vi "fake tool unwired error.vi"(11 "json":string) -> (3 "count":i32)   [LabVIEW 2020, in "MCP Server tests.lvlib"]
doc: "Test fixture tool: counts the items of the JSON object json. The parse error of a json that is not an object appears on an unwired error output, and the VI has automatic error handling enabled, so that a server which runs it without switching that off opens LabVIEW's modal error dialog."
uses:
  MCP Server tests.lvlib
  <vilib>/JDP Science/JSONtext/JSONtext.lvlib
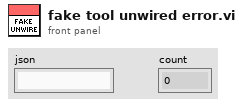
[diagram p1: front panel]
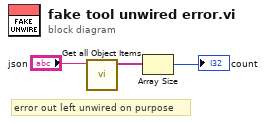
[diagram p0: block diagram]
diagram:
  # "error out left unwired on purpose"
  n1 = call <vilib>:"Get all Object Items.vi"("JSON"="json") -> ("Item Names"=w3:string[])  [unwired: 7 in, 3 out]
  n2 = Array Size(array=w3) -> (size(s)=→"count":i32)
